vi "FRC Strings.vi"() -> ()   [LabVIEW 2023]
panel:
  in  "Initial dashboard project name":string="2027 Dashboard Project"
  in  "Dashboard Title bar":string="Create New FRC Dashboard Project"
  in  "Duplicate project on disk":string="A project named %s, saved at %s, already exists. Do you wish to overwrite the project?"
  in  "Overwrite duplicate project on disk":string="Overwrite project"
  in  "Close duplicate project in memory":string="Close and overwrite project"
  in  "Duplicate project in memory":string="A project named %s, saved at %s, is currently open. Do you wish to close and overwrite the project?"
  in  "Status.Finished":string="Configuring project..."
  in  "cRIO Title bar":string="Create New FRC Robot Project"
  in  "Initial cRIO project name":string="2027 Robot Project"
  # "Other"
  # "Dialogs"
  # "Controls/Indicators"
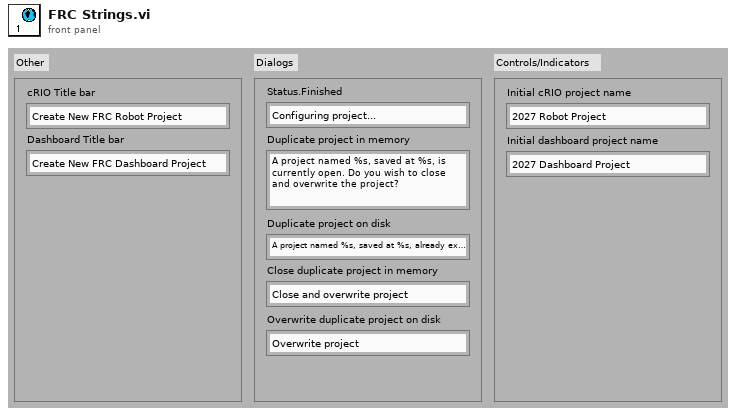
[diagram p1: front panel]
diagram:
